vi "Close.vi"(0 "WebSocket Connection in":refnum<k5>, 1 "timeout ms (5000)":i32=5000, 5 "Send Reason (F)":bool, 7 "Status Code":T1=1000 items=["Normal Closure"=1000, "Going Away"=1001, "Protocol Error"=1002, "Wrong Data Type"=1003, "Reserved 1004"=1004, "Reserved 1005"=1005, "Reserved 1006"=1006, "Non Consistent Data Type"=1007, "Policy Violation"=1008, "Message Too Big"=1009, "Extensions Negotiation Error"=1010, "Unexpected Condition"=1011, "Reserved 1015"=1015], 9 "Reason":string, 11 "error in (no error)":errorcluster, 12 "Mask payload?":bool) -> (4 "WebSocket Connection in":refnum<k5>, 15 "error out":errorcluster)   [LabVIEW 2017, in "LV WebSockets.lvlib"]
doc: "Sends the shutdown opcode to the TCP socket. This VI will run even if an upstream error has occurred.\n\nNote: This does not close the TCP connection as you may want to wait for the shutdown opcode to be received from the client.\nWebSockets 1.6.0.22\nSam Sharp - MediaMongrels Ltd\nCopyright (c) 2016, MediaMongrels Ltd"
uses:
  LV WebSockets.lvlib
  StatusCode.ctl
  Opcode.ctl
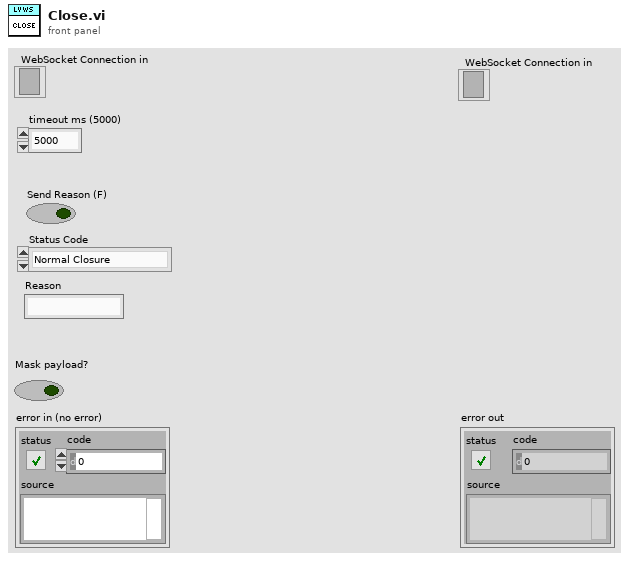
[diagram p1: front panel]
types:
  T1 = typedef "LV WebSockets.lvlib/StatusCode.ctl" = u16
  T2 = typedef "LV WebSockets.lvlib/Opcode.ctl" = enum8{"Continuation Frame", "Text Frame", "Binary Frame", "Reserved 3", "Reserved 4", "Reserved 5", "Reserved 6", "Reserved 7", "Connection Close", "Ping", "Pong", "Reserved B", "Reserved C", "Reserved D", "Reserved F"}
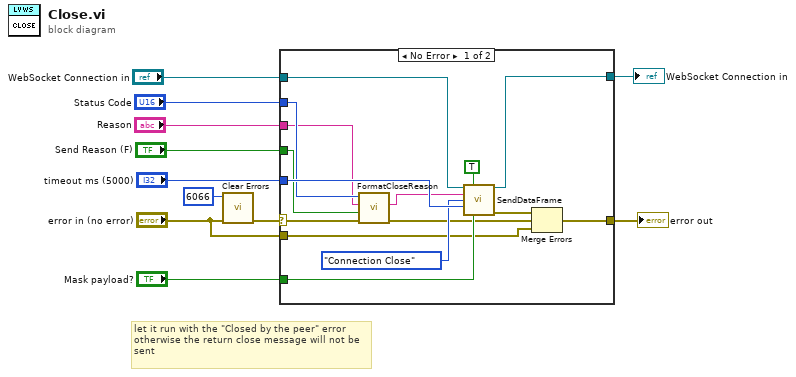
[diagram p0: block diagram]
diagram:
  # "let it run with the \"Closed by the peer\" error otherwise the return close message will not be sent"
  n1 = call <vilib>:"Clear Errors.vi"("error in (no error)"="error in (no error)", "specific error code to clear (0: all)"=6066) -> ("error out"=w2:errorcluster)  [unwired: 4 in, 1 out]
  n2 = case shown="No Error" w2 {
    selector: w2 -> [w14 w28]
    tunnel: [w26 w28] -> w11
    tunnel: [w25 w27] -> w9
    tunnel: "WebSocket Connection in" -> [w24 w27]
    tunnel: "timeout ms (5000)" -> [w23 _]
    tunnel: "Mask payload?" -> [w20 _]
    tunnel: "Status Code" -> [w18 _]
    tunnel: "Reason" -> [w17 _]
    tunnel: "Send Reason (F)" -> [w15 _]
    tunnel: "error in (no error)" -> [w12 _]
    frame No Error {
      n3 = call "FormatCloseReason.vi"("error in (no error)"=w14, "Send Reason (F)"=w15, "Reason"=w17, "Status Code"=w18) -> ("error out"=w13:errorcluster, "Application Data"=w16:string)  [unwired: 5 in]
      n4 = call "SendDataFrame.vi"("WebSocket Connection in"=w24, "Final Frame Bit  (F)"=TRUE ("FIN Bit (F)"), "Data"=w16, "Opcode"=Opcode."Connection Close", "timeout ms (5000)"=w23, "Mask payload?"=w20) -> ("WebSocket Connection out"=w25:refnum<k5>, "error out"=w21:errorcluster)  [unwired: 8 in]
      n5 = Merge Errors(w21, w13, w12) -> (w26:errorcluster)
    }
    frame Error {
    }
  }
  "WebSocket Connection in" <- w9
  "error out" <- w11
